vi "ZM-TST-protocol.vi"() -> (0 "error out":errorcluster, 3 "Pass":bool)   [LabVIEW 2020, in "ZM-TST-tests.lvlib"]
doc: "T4, test of the file logger in a fresh temp folder under output: init creates the folder, each published package lands as one line in the file of its type, a later publish appends, and the bare protocol and a multi protocol holding it return 5000. Pass = AND of the seven checks. Side effect: three JSONL files in the temp folder."
uses:
  ZM-TST-tests.lvlib
  protocol/ZM-CP-FL-file_logger/ZM-CP-FL-file_logger/ZM-CP-FL-file_logger.lvclass
  protocol/ZM-CP-communication_protocol/ZM-CP-communication_protocol/ZM-CP-communication_protocol.lvclass
  common/ZM-PC-packages/ZM-PC-package/ZM-PC-package.lvclass
  protocol/ZM-CP-MX-multi_protocol/ZM-CP-MX-multi_protocol/ZM-CP-MX-multi_protocol.lvclass
  common/ZM-PC-packages/ZM-PC-TP-test_package/ZM-PC-TP-test_package.lvclass
  common/ZM-PC-packages/ZM-PC-EP-error_package/ZM-PC-EP-error_package.lvclass
panel:
  out "mx_placeholder_ok":bool
  out "close_ok":bool
  out "placeholder_ok":bool
  out "append_ok":bool
  out "lines_ok":bool
  out "files_ok":bool
  out "init_ok":bool
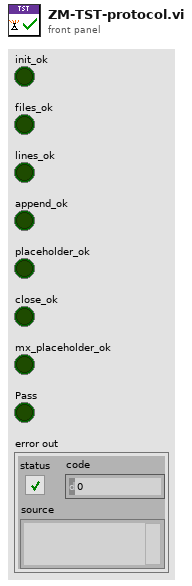
[diagram p1: front panel]
types:
  T1 = cluster{"timestamp":string, "type":string, "destination":string, "data":cluster{"sender":string, "code":i32, "source":string}}
  T2 = cluster{"timestamp":string, "type":string, "destination":string}
  T3 = cluster{"timestamp":string, "type":string, "destination":string, "data":cluster{"temperature_c":dbl, "sample_index":i32, "duty_percent":u8, "sensor_ok":bool, "status":string}}
  T4 = cluster{"temperature_c":dbl, "sample_index":i32, "duty_percent":u8, "sensor_ok":bool, "status":string}
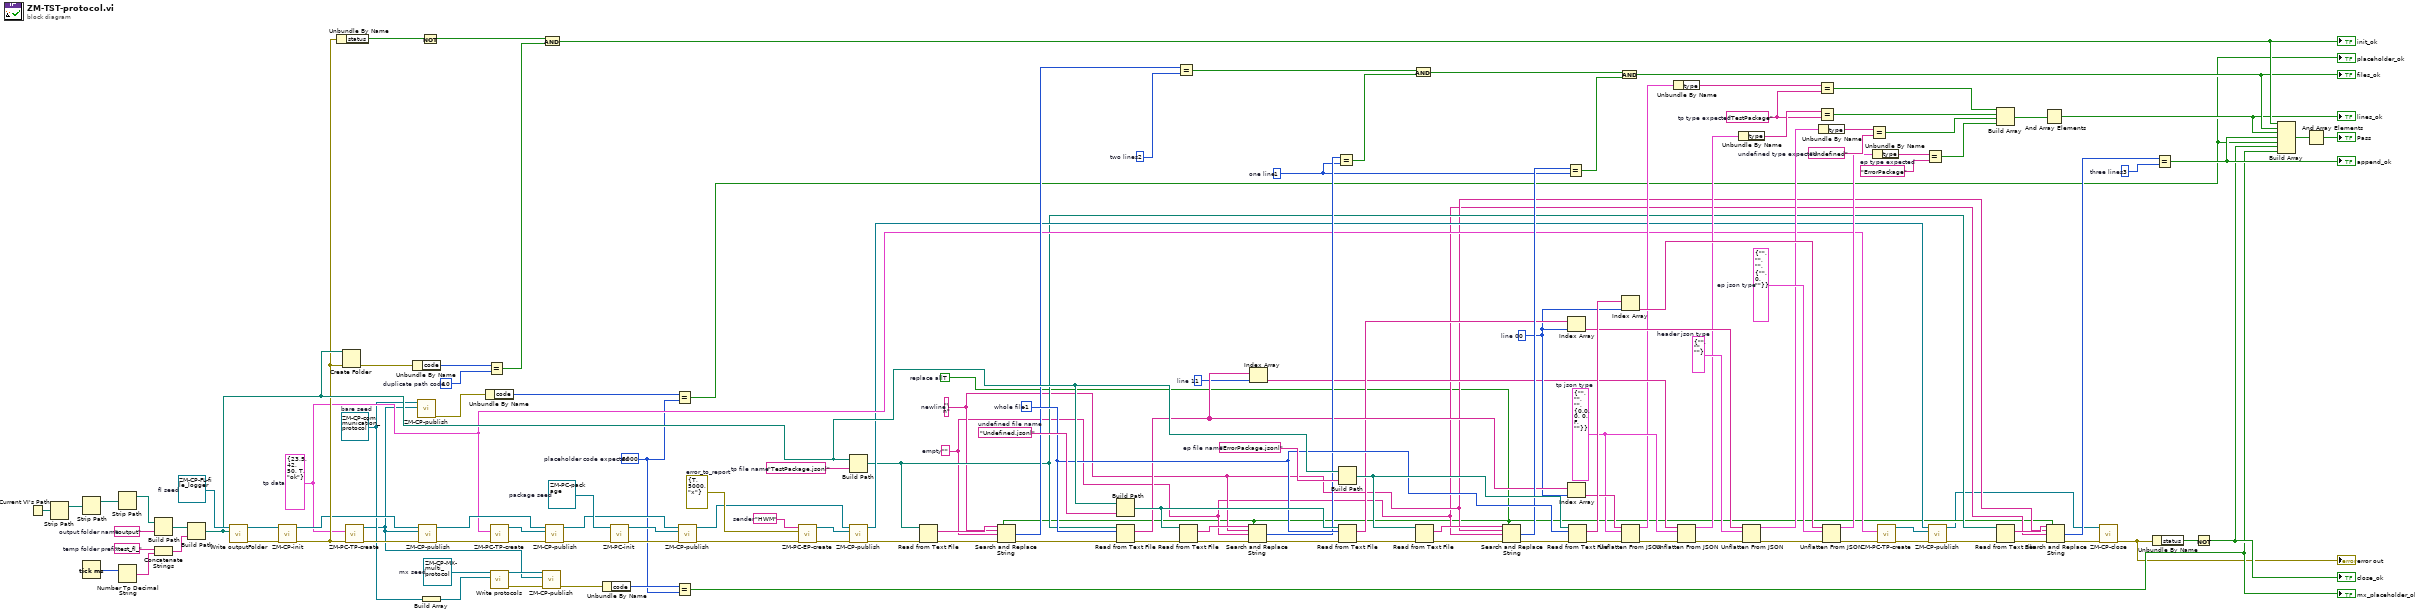
[diagram p0: block diagram]
diagram:
  w69 = 1  # line 1
  w66 = 0  # line 0
  w25 = 3  # three lines
  w75 = 1  # one line
  w78 = 2  # two lines
  w14 = 5000  # placeholder code expected
  w115 = 10  # duplicate path code
  w81 = -1  # whole file
  w27 = TRUE  # replace all
  w29 = ""  # empty
  w30 = "\n"  # newline
  w56 = T1 {"timestamp"="", "type"="", "destination"="", "data"={"sender"="", "code"=0, "source"=""}}  # ep json type
  w59 = T2 {"timestamp"="", "type"="", "destination"=""}  # header json type
  w62 = T3 {"timestamp"="", "type"="", "destination"="", "data"={"temperature_c"=0.0, "sample_index"=0, "duty_percent"=0, "sensor_ok"=FALSE, "status"=""}}  # tp json type
  w44 = "ErrorPackage"  # ep type expected
  w47 = "Undefined"  # undefined type expected
  w50 = "TestPackage"  # tp type expected
  w123 = "ErrorPackage.jsonl"  # ep file name
  w124 = "Undefined.jsonl"  # undefined file name
  w125 = "TestPackage.jsonl"  # tp file name
  w134 = "test_fl_"  # temp folder prefix
  w128 = "output"  # output folder name
  w99 = errorcluster {"status"=TRUE, "code"=5000, "source"="x"}  # error_to_report
  w100 = "HWM"  # sender
  w38 = T4 {"temperature_c"=23.5, "sample_index"=42, "duty_percent"=50, "sensor_ok"=TRUE, "status"="ok"}  # tp data
  w21 = refnum<class "ZM-CP-MX-multi_protocol.lvclass"> refnum  # mx seed
  w105 = refnum<class "ZM-PC-package.lvclass"> refnum  # package seed
  w22 = refnum<class "ZM-CP-communication_protocol.lvclass"> refnum  # bare seed
  w122 = refnum<class "ZM-CP-FL-file_logger.lvclass"> refnum  # fl seed
  n1 = Current VI's Path() -> (path=w132:path)
  n2 = Strip Path(path=w132) -> (stripped path=w131:path)  [unwired: 1 out]
  n3 = Strip Path(path=w131) -> (stripped path=w130:path)  [unwired: 1 out]
  n4 = Tick Count (ms)() -> (millisecond timer value=w135:u32)
  n5 = Strip Path(path=w130) -> (stripped path=w129:path)  [unwired: 1 out]
  n6 = Number To Decimal String(number=w135) -> (decimal integer string=w133:string)  [unwired: 1 in]
  n7 = Build Path(base path=w129, name or relative path=w128) -> (appended path=w127:path)
  n8 = Concatenate Strings(w134, w133) -> (w126:string)
  n9 = Build Path(base path=w127, name or relative path=w126) -> (appended path=w118:path)
  n10 = call "Write outputFolder.vi"("outputFolder"=w118, "ZM-CP-FL-file_logger in"=w122) -> ("error out"=w120:errorcluster, "ZM-CP-FL-file_logger out"=w121:refnum<class "ZM-CP-FL-file_logger.lvclass">)  [unwired: 8 in]
  n11 = call-dynamic "ZM-CP-init.vi"("error in (no error)"=w120, "ZM-CP-FL-file_logger in"=w121) -> ("error out"=w112:errorcluster, "ZM-CP-FL-file_logger out"=w111:refnum<class "ZM-CP-FL-file_logger.lvclass">)  [unwired: 8 in]
  n12 = Unbundle By Name(w112) -> ("status"=w119:bool)
  n13 = Create Folder(path (use dialog)=w118, error in=w112) -> (error out=w117:errorcluster)  [unwired: 1 in, 2 out]
  n14 = call "ZM-PC-TP-create.vi"("error in (no error)"=w112, "data"=w38) -> ("error out"=w110:errorcluster, "package"=w18:refnum<class "ZM-PC-TP-test_package.lvclass">)  [unwired: 8 in]
  n15 = Unbundle By Name(w117) -> ("code"=w116:i32)
  n16 = call-dynamic "ZM-CP-publish.vi"("package"=w18, "ZM-CP-communication_protocol in"=w22) -> ("error out"=w24:errorcluster)  [unwired: 8 in, 1 out]
  n17 = call-dynamic "ZM-CP-publish.vi"("error in (no error)"=w110, "package"=w18, "ZM-CP-FL-file_logger in"=w111) -> ("error out"=w109:errorcluster, "ZM-CP-FL-file_logger out"=w108:refnum<class "ZM-CP-FL-file_logger.lvclass">)  [unwired: 7 in]
  n18 = Not(x=w119) -> (.not. x?=w114:bool)
  n19 = Build Array(w22) -> (w20:refnum<class "ZM-CP-communication_protocol.lvclass">[])
  n20 = Unbundle By Name(w24) -> ("code"=w23:i32)
  n21 = Equal?(x=w116, y=w115) -> (x = y?=w113:bool)
  n22 = call "ZM-PC-TP-create.vi"("error in (no error)"=w109, "data"=w38) -> ("error out"=w106:errorcluster, "package"=w107:refnum<class "ZM-PC-TP-test_package.lvclass">)  [unwired: 8 in]
  n23 = call "Write protocols.vi"("ZM-CP-MX-PROTOCOLS"=w20, "ZM-CP-MX-multi_protocol in"=w21) -> ("error out"=w17:errorcluster, "ZM-CP-MX-multi_protocol out"=w19:refnum<class "ZM-CP-MX-multi_protocol.lvclass">)  [unwired: 8 in]
  n24 = call-dynamic "ZM-CP-publish.vi"("error in (no error)"=w17, "package"=w18, "ZM-CP-MX-multi_protocol in"=w19) -> ("error out"=w16:errorcluster)  [unwired: 7 in, 1 out]
  n25 = And(x=w114, y=w113) -> (x .and. y?=w9:bool)
  "init_ok" <- w9
  n26 = call-dynamic "ZM-CP-publish.vi"("error in (no error)"=w106, "package"=w107, "ZM-CP-FL-file_logger in"=w108) -> ("error out"=w104:errorcluster, "ZM-CP-FL-file_logger out"=w103:refnum<class "ZM-CP-FL-file_logger.lvclass">)  [unwired: 7 in]
  n27 = Unbundle By Name(w16) -> ("code"=w15:i32)
  n28 = call-dynamic "ZM-PC-init.vi"("error in (no error)"=w104, "ZM-PC-package in"=w105) -> ("error out"=w101:errorcluster, "ZM-PC-package out"=w102:refnum<class "ZM-PC-package.lvclass">)  [unwired: 8 in]
  n29 = Equal?(x=w23, y=w14) -> (x = y?=w5:bool)
  "placeholder_ok" <- w5
  n30 = Equal?(x=w15, y=w14) -> (x = y?=w3:bool)
  "mx_placeholder_ok" <- w3
  n31 = call-dynamic "ZM-CP-publish.vi"("error in (no error)"=w101, "package"=w102, "ZM-CP-FL-file_logger in"=w103) -> ("error out"=w98:errorcluster, "ZM-CP-FL-file_logger out"=w97:refnum<class "ZM-CP-FL-file_logger.lvclass">)  [unwired: 7 in]
  n32 = call "ZM-PC-EP-create.vi"("error in (no error)"=w98, "error_to_report"=w99, "sender"=w100) -> ("error out"=w95:errorcluster, "package"=w96:refnum<class "ZM-PC-EP-error_package.lvclass">)  [unwired: 7 in]
  n33 = Build Path(base path=w118, name or relative path=w125) -> (appended path=w33:path)
  n34 = call-dynamic "ZM-CP-publish.vi"("error in (no error)"=w95, "package"=w96, "ZM-CP-FL-file_logger in"=w97) -> ("error out"=w94:errorcluster, "ZM-CP-FL-file_logger out"=w36:refnum<class "ZM-CP-FL-file_logger.lvclass">)  [unwired: 7 in]
  n35 = Read from Text File(file (use dialog)=w33, error in=w94) -> (text=w93:string, error out=w92:errorcluster)  [unwired: 2 in, 2 out]
  n36 = Search and Replace String(replace all?=w27, input string=w93, search string=w30, replace string=w29, error in=w92) -> (number of replacements=w79:i32, error out=w91:errorcluster)  [unwired: 3 in, 2 out]
  n37 = Build Path(base path=w118, name or relative path=w124) -> (appended path=w87:path)
  n38 = Read from Text File(file (use dialog)=w33, count=w81, error in=w91) -> (text=w70:string[], error out=w90:errorcluster)  [unwired: 1 in, 2 out]
  n39 = Equal?(x=w79, y=w78) -> (x = y?=w74:bool)
  n40 = Read from Text File(file (use dialog)=w87, error in=w90) -> (text=w89:string, error out=w88:errorcluster)  [unwired: 2 in, 2 out]
  n41 = Search and Replace String(replace all?=w27, input string=w89, search string=w30, replace string=w29, error in=w88) -> (number of replacements=w77:i32, error out=w86:errorcluster)  [unwired: 3 in, 2 out]
  n42 = Index Array(array=w70, index=w69) -> (element=w63:string)
  n43 = Equal?(x=w77, y=w75) -> (x = y?=w73:bool)
  n44 = Build Path(base path=w118, name or relative path=w123) -> (appended path=w82:path)
  n45 = Read from Text File(file (use dialog)=w87, count=w81, error in=w86) -> (text=w68:string[], error out=w85:errorcluster)  [unwired: 1 in, 2 out]
  n46 = And(x=w74, y=w73) -> (x .and. y?=w72:bool)
  n47 = Read from Text File(file (use dialog)=w82, error in=w85) -> (text=w84:string, error out=w83:errorcluster)  [unwired: 2 in, 2 out]
  n48 = Search and Replace String(replace all?=w27, input string=w84, search string=w30, replace string=w29, error in=w83) -> (number of replacements=w76:i32, error out=w80:errorcluster)  [unwired: 3 in, 2 out]
  n49 = Equal?(x=w76, y=w75) -> (x = y?=w71:bool)
  n50 = Index Array(array=w68, index=w66) -> (element=w60:string)
  n51 = Index Array(array=w70, index=w66) -> (element=w65:string)
  n52 = Read from Text File(file (use dialog)=w82, count=w81, error in=w80) -> (text=w67:string[], error out=w64:errorcluster)  [unwired: 1 in, 2 out]
  n53 = And(x=w72, y=w71) -> (x .and. y?=w8:bool)
  "files_ok" <- w8
  n54 = Index Array(array=w67, index=w66) -> (element=w57:string)
  n55 = Unflatten From JSON(JSON string=w65, type and defaults=w62, error in (no error)=w64) -> (value=w54:T3, error out=w61:errorcluster)  [unwired: 4 in]
  n56 = Unbundle By Name(w54) -> ("type"=w53:string)
  n57 = Unflatten From JSON(JSON string=w63, type and defaults=w62, error in (no error)=w61) -> (value=w52:T3, error out=w58:errorcluster)  [unwired: 4 in]
  n58 = Unbundle By Name(w52) -> ("type"=w51:string)
  n59 = Unflatten From JSON(JSON string=w60, type and defaults=w59, error in (no error)=w58) -> (value=w49:T2, error out=w55:errorcluster)  [unwired: 4 in]
  n60 = Equal?(x=w53, y=w50) -> (x = y?=w43:bool)
  n61 = Equal?(x=w51, y=w50) -> (x = y?=w42:bool)
  n62 = Unbundle By Name(w49) -> ("type"=w48:string)
  n63 = Unflatten From JSON(JSON string=w57, type and defaults=w56, error in (no error)=w55) -> (value=w46:T1, error out=w37:errorcluster)  [unwired: 4 in]
  n64 = Equal?(x=w48, y=w47) -> (x = y?=w41:bool)
  n65 = Unbundle By Name(w46) -> ("type"=w45:string)
  n66 = call "ZM-PC-TP-create.vi"("error in (no error)"=w37, "data"=w38) -> ("error out"=w34:errorcluster, "package"=w35:refnum<class "ZM-PC-TP-test_package.lvclass">)  [unwired: 8 in]
  n67 = Equal?(x=w45, y=w44) -> (x = y?=w40:bool)
  n68 = call-dynamic "ZM-CP-publish.vi"("error in (no error)"=w34, "package"=w35, "ZM-CP-FL-file_logger in"=w36) -> ("error out"=w32:errorcluster, "ZM-CP-FL-file_logger out"=w13:refnum<class "ZM-CP-FL-file_logger.lvclass">)  [unwired: 7 in]
  n69 = Build Array(w43, w42, w41, w40) -> (w39:bool[])
  n70 = Read from Text File(file (use dialog)=w33, error in=w32) -> (text=w31:string, error out=w28:errorcluster)  [unwired: 2 in, 2 out]
  n71 = And Array Elements(Boolean array=w39) -> (logical AND=w7:bool)
  "lines_ok" <- w7
  n72 = Search and Replace String(replace all?=w27, input string=w31, search string=w30, replace string=w29, error in=w28) -> (number of replacements=w26:i32, error out=w12:errorcluster)  [unwired: 3 in, 2 out]
  n73 = call-dynamic "ZM-CP-close.vi"("error in (no error)"=w12, "ZM-CP-communication_protocol in"=w13) -> ("error out"=w1:errorcluster)  [unwired: 8 in, 1 out]
  "error out" <- w1
  n74 = Unbundle By Name(w1) -> ("status"=w11:bool)
  n75 = Equal?(x=w26, y=w25) -> (x = y?=w6:bool)
  "append_ok" <- w6
  n76 = Not(x=w11) -> (.not. x?=w4:bool)
  "close_ok" <- w4
  n77 = Build Array(w9, w8, w7, w6, w5, w4, w3) -> (w10:bool[])
  n78 = And Array Elements(Boolean array=w10) -> (logical AND=→"Pass":bool)
